vi "set Gate Source Type.vi"(8 "error in (no error)":errorcluster, 10 "Gate Source":T1(ring), 11 "Keysight 9020A in":refnum<class "Keysight 9020A.lvclass">) -> (0 "error out":errorcluster, 3 "Keysight 9020A out":refnum<class "Keysight 9020A.lvclass">)   [LabVIEW 2023, in "Spectrum Analyzer.lvlib" / "Keysight 9020A.lvclass"]
uses:
  Keysight 9020A.lvclass
  Keysight 9020A.lvclass/Keysight 9020A.ctl
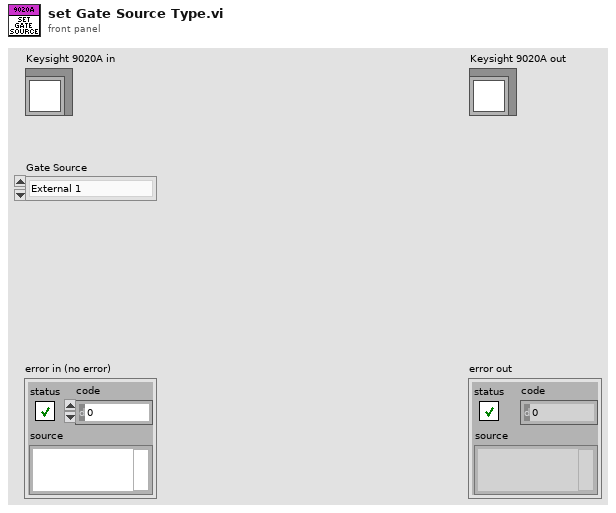
[diagram p1: front panel]
types:
  T1 = enum16{"External 1", "External 2", "Line", "Frame", "RF Burst", "TV", "PXI"}
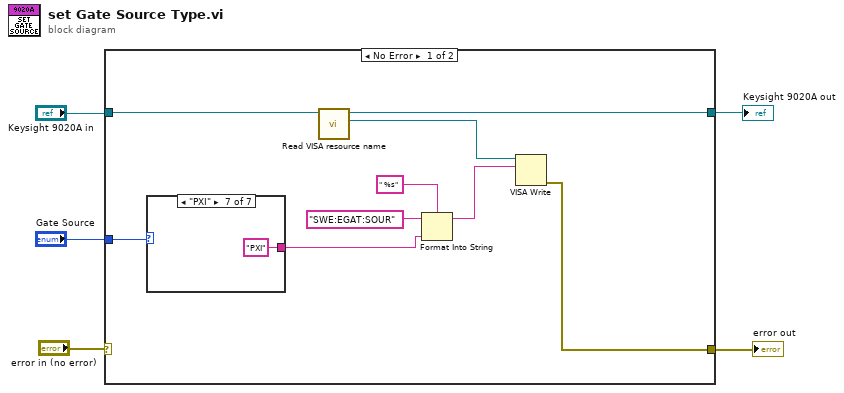
[diagram p0: block diagram]
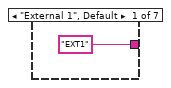
[diagram p2: hidden frame]
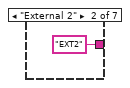
[diagram p3: hidden frame]
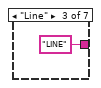
[diagram p4: hidden frame]
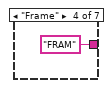
[diagram p5: hidden frame]
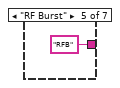
[diagram p6: hidden frame]
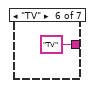
[diagram p7: hidden frame]
diagram:
  n1 = case shown="No Error" "error in (no error)" {
    selector: "error in (no error)" -> [_ w22]
    tunnel: "Keysight 9020A in" -> [w9 w23]
    tunnel: [w14 w23] -> w4
    tunnel: [w10 w22] -> w1
    tunnel: "Gate Source" -> [w8 _]
    frame No Error {
      n2 = case shown="\"PXI\"" w8 {
        tunnel: ["EXT1" "EXT2" "LINE" "FRAM" "RFB" "TV" "PXI"] -> w7
        frame "External 1", Default {
        }
        frame "External 2" {
        }
        frame "Line" {
        }
        frame "Frame" {
        }
        frame "RF Burst" {
        }
        frame "TV" {
        }
        frame "PXI" {
        }
      }
      n3 = call "Read VISA resource name.vi"("Keysight 9020A in"=w9) -> ("VISA resource name"=w12:refnum<visa-resource-name>, "Keysight 9020A out"=w14:refnum<class "Keysight 9020A.lvclass">)  [unwired: 8 in, 1 out]
      n4 = Format Into String(format string=" %s", initial string="SWE:EGAT:SOUR" ("string"), w7) -> (resulting string=w11:string)  [unwired: 1 in, 1 out]
      n5 = VISA Write(VISA resource name=w12, write buffer=w11) -> (error out=w10:errorcluster)  [unwired: 1 in, 2 out]
    }
    frame Error {
    }
  }
  "error out" <- w1
  "Keysight 9020A out" <- w4
